vi "Registry_Get_Snapshot.vi"(8 "error in (no error)":errorcluster={"status"=FALSE, "code"=0, "source"="\"\""}, 10 "time boundary":string, 11 "Parameter ID set":string) -> (0 "error out":errorcluster={"status"=FALSE, "code"=0, "source"="\"\""}, 2 "status ok":bool, 3 "ParameterSnapshot":string)   [LabVIEW 2026]
doc: "INTENT: Return coherent evaluation data. LOGIC: Copy required values and source timestamps in one registry service transaction."
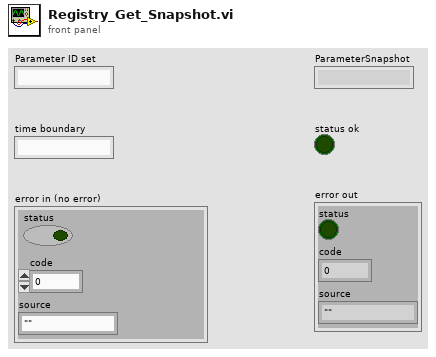
[diagram p1: front panel]
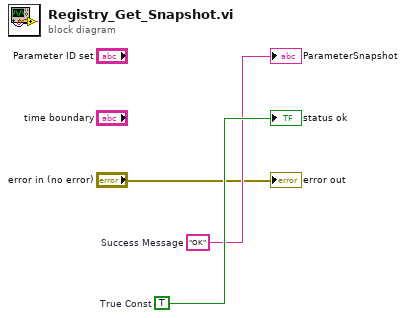
[diagram p0: block diagram]
diagram:
  w3 = TRUE  # True Const
  w2 = "OK"  # Success Message
  "ParameterSnapshot" <- w2
  "status ok" <- w3
  "error out" <- "error in (no error)"
